vi "RichToFlatcif_can_reader_nixnet_InterfaceBlink.vi"(5 "OutputClusterType":T1, 11 "InputCluster":T2) -> (3 "OutputCluster":T1)   [LabVIEW 2021, in "CanReaderNixnet_client.lvlib"]
uses:
  CanReaderNixnet_client.lvlib
  cif_can_reader_nixnet_InterfaceBlink.ctl
  cif_can_reader_nixnet_InterfaceBlink_Flat.ctl
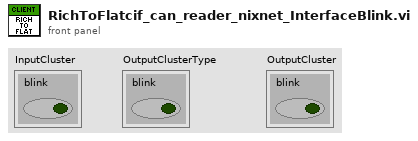
[diagram p1: front panel]
types:
  T1 = typedef "CanReaderNixnet_client.lvlib/cif_can_reader_nixnet_InterfaceBlink_Flat.ctl" = cluster{"blink":bool}
  T2 = typedef "CanReaderNixnet_client.lvlib/cif_can_reader_nixnet_InterfaceBlink.ctl" = cluster{"blink":bool}
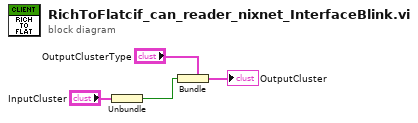
[diagram p0: block diagram]
diagram:
  n1 = Unbundle "Unbundle"("InputCluster") -> ("blink"=w1:bool)
  n2 = Bundle "Bundle"(cluster="OutputClusterType", "blink"=w1) -> (→"OutputCluster":T1)
